vi "Create CIF Subscriber.vi"(6 "Timeout (ms)":u32=5000, 8 "error in (no error)":errorcluster, 10 "Universal":bool, 11 "CIF Pcap Subscriber Configuration":T2) -> (0 "error out":errorcluster, 3 "CIF Subscriber Refnum":T1 {"refnum" format="%.0x"})   [LabVIEW 2021, in "Iceoryx.lvlib"]
doc: "Create an iceoryx subscriber. This can create either a backpressure or best effort subscriber. Best effort will overflow if the subscribers don't keep up, backpressure which will block the writer. \n\nSubscriber configuration:\n<B>Name:</B> Shared between multiple queue streams from the same source\n<B>Topic:</B> Unique name for this queue stream under the source name. Name/topic must be unique in the system\n<B>Link Type:</B> pcap Link Type used for subscriber type checks\n<B>Backpressure:</B> Sets if the subscriber will provide backpressure\n\n<B>Universal:</B> Sets the subscriber to skip type check"
uses:
  Iceoryx.lvlib
  typedef/CIF Pcap Subscriber Configuration.ctl
  Refnum/Typedef/CIF Subscriber Refnum.ctl
  typedef/Errors.ctl
  SubVIs/Add Error Core.vi
  <vilib>/CIF Foundation/CIF Utilities/File/SubVIs/File Not Found Error Core.vi
  SubVIs/Convert Error Core.vi
  <vilib>/CIF Foundation/CIF Utilities/File/File_CIF_U.lvlib
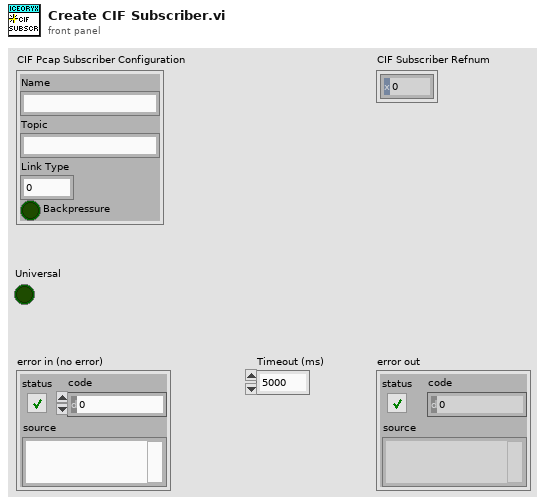
[diagram p1: front panel]
types:
  T1 = typedef "Iceoryx.lvlib/CIF Subscriber Refnum.ctl" = cluster{"refnum":u64, "CIF Sub":enum8{"cifsub"}}
  T2 = typedef "Iceoryx.lvlib/CIF Pcap Subscriber Configuration.ctl" = cluster{"Name":string, "Topic":string, "Link Type":u32, "Backpressure":bool}
  T3 = typedef "Iceoryx.lvlib/Errors.ctl" = enum16{"Unsupported Type", "Empty Name", "Cluster Name"}
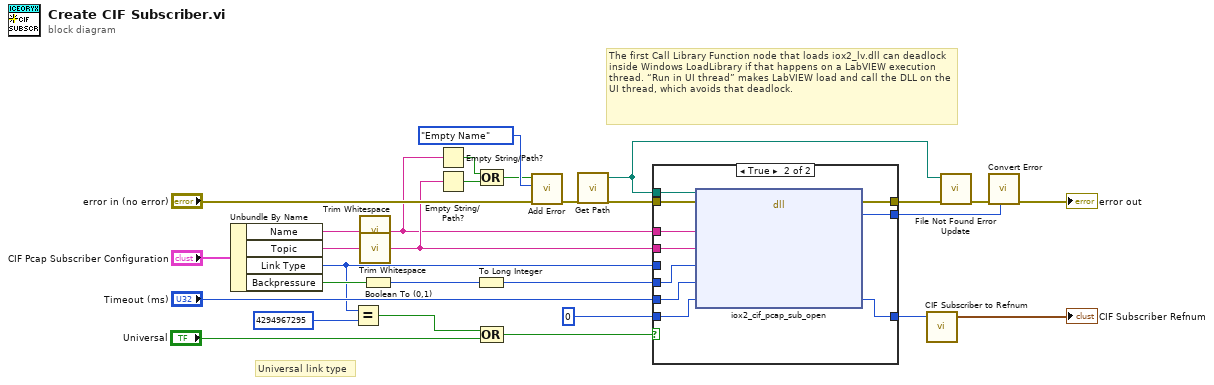
[diagram p0: block diagram]
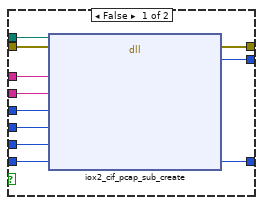
[diagram p2: hidden frame]
diagram:
  # "Universal link type"
  # "The first Call Library Function node that loads iox2_lv.dll can deadlock inside Windows LoadLibrary if that happens on a LabVIEW execution thread. “Run in UI thread” makes LabVIEW load and call the DLL on the UI thread, which avoids that deadlock."
  n1 = Unbundle By Name("CIF Pcap Subscriber Configuration") -> ("Name"=w14:string, "Topic"=w13:string, "Link Type"=w5:u32, "Backpressure"=w11:bool)
  n2 = Equal?(x=w5, y=u32 4294967295 ("t")) -> (x = y?=w2:bool)
  n3 = call <vilib>:"Trim Whitespace.vi"("string"=w14) -> ("trimmed string"=w15:string)  [unwired: 1 in]
  n4 = call <vilib>:"Trim Whitespace.vi"("string"=w13) -> ("trimmed string"=w16:string)  [unwired: 1 in]
  n5 = Boolean To (0,1)(Boolean=w11) -> (0, 1=w12:i16)
  n6 = Empty String/Path?(string/path=w15) -> (empty?=w18:bool)
  n7 = Empty String/Path?(string/path=w16) -> (empty?=w19:bool)
  n8 = To Long Integer(number=w12) -> (32bit integer=w10:i32)
  n9 = Compound Arithmetic op=OR(w18, w19) -> (w17:bool)
  n10 = Compound Arithmetic op=OR(w2, "Universal") -> (w1:bool)
  n11 = call "Add Error.vi"("error in (no error)"="error in (no error)", "Error"=Errors."Empty Name", "Insert Error"=w17) -> ("error out"=w8:errorcluster)  [unwired: 8 in]
  n12 = call "Get Path.vi"() -> ("libiox2_cif path"=w25:path)  [unwired: 4 in]
  n13 = case shown="True" w1 {
    tunnel: [w39 w49] -> w7
    tunnel: "Timeout (ms)" -> [w38 w41]
    tunnel: u64 0 ("writer") -> [w37 w40]
    tunnel: w25 -> [w36 w48]
    tunnel: [w35 w47] -> w24
    tunnel: [w34 w46] -> w23
    tunnel: w16 -> [w33 w45]
    tunnel: w15 -> [w32 w44]
    tunnel: w10 -> [w31 w42]
    tunnel: w8 -> [w30 w43]
    tunnel: w5 -> [w29 _]
    frame False {
      n14 = dll-call lib="D:/dev/iceoryx2_lvwrapper/dist/iox2_cif.dll" fn="iox2_cif_pcap_sub_create"(path in=w36, error in=w30, "name"=w32, "topic"=w33, "link_type"=w29, "use_backpressure"=w31, "timeout_ms"=w38, "reader"=w37) -> (error out=w35:errorcluster, "return type"=w34:i32, "reader"=w39:u64)  [unwired: 6 in, 1 out]
    }
    frame True {
      n15 = dll-call lib="D:/dev/iceoryx2_lvwrapper/dist/iox2_cif.dll" fn="iox2_cif_pcap_sub_open"(path in=w48, error in=w43, "name"=w44, "topic"=w45, "use_backpressure"=w42, "timeout_ms"=w41, "reader"=w40) -> (error out=w47:errorcluster, "return type"=w46:i32, "reader"=w49:u64)  [unwired: 5 in, 1 out]
    }
  }
  n16 = call "CIF Subscriber to Refnum.vi"("CIF Subscriber U64"=w7) -> ("CIF Subscriber Refnum"=→"CIF Subscriber Refnum":T1)  [unwired: 4 in]
  n17 = call <vilib>:"File Not Found Error Update.vi"("error in"=w24, "path in"=w25) -> ("error out"=w26:errorcluster)  [unwired: 9 in]
  n18 = call "Convert Error.vi"("return type"=w23, "error in (no error)"=w26) -> ("error out"=→"error out":errorcluster)  [unwired: 9 in]
